vi "Stop Triggered Acq.vi"(8 "error in (no error)":errorcluster, 11 "DAQ Timed SPIM in":refnum<class "DAQ Timed SPIM.lvclass">) -> (0 "error out":errorcluster, 3 "DAQ Timed SPIM out":refnum<class "DAQ Timed SPIM.lvclass">)   [LabVIEW 2020, in "DAQ Timed SPIM.lvlib" / "DAQ Timed SPIM.lvclass"]
uses:
  DAQ Timed SPIM.lvclass
  DAQ Timed SPIM.lvclass/DAQ Timed SPIM.ctl
  <vilib>/Utility/error.llb/DialogType.ctl
  <vilib>/ActorFramework/Message Enqueuer/Message Enqueuer.lvclass/Message Enqueuer.ctl
  <vilib>/DAQmx/write.llb/DAQmx Write (Digital 2D U8 NChan NSamp).vi
  <vilib>/DAQmx/write.llb/DAQmx Write (Analog 2D DBL NChan NSamp).vi
  <vilib>/ActorFramework/Message Enqueuer/Enqueue.vi
  Abstract DAQ Triggered Actor Messages/Stop Msg/Stop Acq Msg.lvclass
  C:/Program Files/National Instruments/LabVIEW 2020/vi.lib/ActorFramework/Message/Message.lvclass
  <vilib>/DAQmx/miscellaneous.llb/DAQmx Fill In Error Info.vi
  <vilib>/ActorFramework/Message Priority Queue/Priority Enqueue.vi
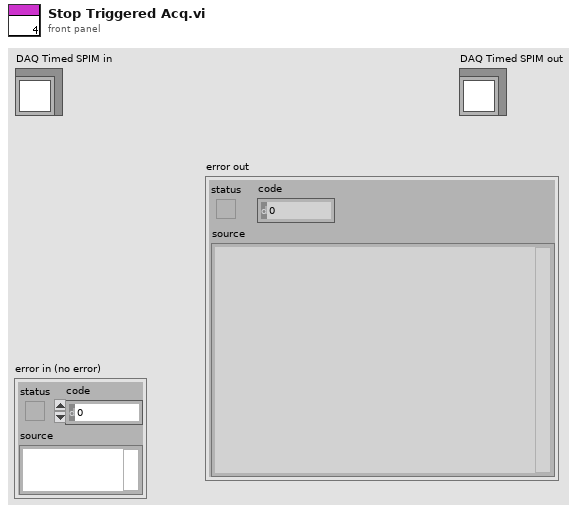
[diagram p1: front panel]
types:
  T1 = typedef "DialogType.ctl" = u16
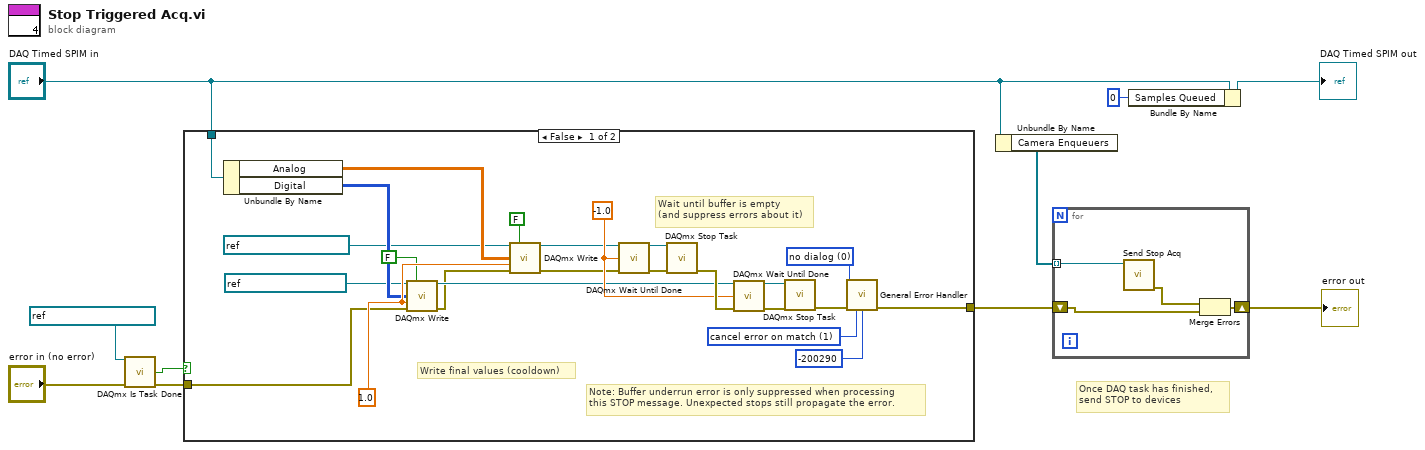
[diagram p0: block diagram]
diagram:
  # "Once DAQ task has finished,\nsend STOP to devices"
  n1 = call <vilib>:"DAQmx Is Task Done.vi"("task/channels in"=refnum<k21> "SPIM_Analog_Task", "error in"="error in (no error)") -> ("task done?"=w6:bool, "error out"=w7:errorcluster)  [unwired: 11 in, 1 out]
  n2 = case shown="False" w6 {
    tunnel: w7 -> [w18 w35]
    tunnel: [w17 w35] -> w4
    tunnel: "DAQ Timed SPIM in" -> [w16 _]
    frame False {
      w19 = 1.0 ("timeout")
      w29 = T1 0 items=["no dialog", "OK message", "continue or stop message", "OK message + warnings", "continue/stop + warnings"] ("type of dialog (OK msg:1)")
      w30 = 1 items=["no exception", "cancel error on match", "set error on match"] ("[exception action] (none:0)")
      w25 = -1.0 ("timeout (sec)")
      # "Write final values (cooldown)"
      # "Note: Buffer underrun error is only suppressed when processing\nthis STOP message. Unexpected stops still propagate the error."
      # "Wait until buffer is empty\n(and suppress errors about it)"
      n3 = Unbundle By Name(w16) -> ("Analog"=w14:dbl[][], "Digital"=w15:u8[][])
      n4 = call-poly <vilib>:"DAQmx Write.vi"("task/channels in"=refnum<k21> "SPIM_Digital_Task", "auto start"=FALSE, "data"=w15, "timeout"=w19, "error in"=w18) -> ("task out"=w24:refnum<k21>, "error out"=w22:errorcluster)  [unwired: 8 in, 1 out]
      n5 = call-poly <vilib>:"DAQmx Write.vi"("task/channels in"=refnum<k21> "SPIM_Analog_Task", "auto start"=FALSE, "data"=w14, "timeout"=w19, "error in"=w22) -> ("task out"=w23:refnum<k21>, "error out"=w21:errorcluster)  [unwired: 8 in, 1 out]
      n6 = call <vilib>:"DAQmx Wait Until Done.vi"("task/channels in"=w23, "timeout (sec)"=w25, "error in"=w21) -> ("task out"=w34:refnum<k21>, "error out"=w33:errorcluster)  [unwired: 11 in]
      n7 = call <vilib>:"DAQmx Stop Task.vi"("task/channels in"=w34, "error in"=w33) -> ("error out"=w26:errorcluster)  [unwired: 12 in, 1 out]
      n8 = call <vilib>:"DAQmx Wait Until Done.vi"("task/channels in"=w24, "timeout (sec)"=w25, "error in"=w26) -> ("task out"=w28:refnum<k21>, "error out"=w27:errorcluster)  [unwired: 11 in]
      n9 = call <vilib>:"DAQmx Stop Task.vi"("task/channels in"=w28, "error in"=w27) -> ("error out"=w32:errorcluster)  [unwired: 12 in, 1 out]
      n10 = call <vilib>:"General Error Handler.vi"("type of dialog (OK msg:1)"=w29, "error in (no error)"=w32, "[exception action] (none:0)"=w30, "[exception code]"=-200290) -> ("error out"=w17:errorcluster)  [unwired: 7 in, 4 out]
    }
    frame True {
    }
  }
  n11 = Unbundle By Name("DAQ Timed SPIM in") -> ("Camera Enqueuers"=w10:refnum<class "Message Enqueuer.lvclass">[])
  n12 = for {
    tunnel: w10 -> [w37] mode=indexing
    shift-right: [w39] -> w3
    shift-left: w4 -> [w38]
    n13 = call "Send Stop Acq.vi"("Message Enqueuer"=w37) -> ("error out"=w36:errorcluster)  [unwired: 9 in, 1 out]
    n14 = Merge Errors(w36, w38) -> (w39:errorcluster)
  }
  "error out" <- w3
  n15 = Bundle By Name(cluster="DAQ Timed SPIM in", "Samples Queued"=0) -> (→"DAQ Timed SPIM out":refnum<class "DAQ Timed SPIM.lvclass">)
